vi "FRC Create Project.vi"(0 "Project folder":path, 1 "Project name":string, 2 "Team number":string, 3 "error in":errorcluster, 4 "frc project type":T1) -> (5 "proceed?":bool, 6 "error out":errorcluster)   [LabVIEW 2027]
uses:
  <resource>/plugins/NewDialogFiles/ProjectWizards/FRC/frc project type.ctl
  <vilib>/Utility/Symbolic Paths/Symbolic Path ID--enum.ctl
  <resource>/plugins/NewDialogFiles/ProjectWizards/FRC/FRC Strings.vi
  <vilib>/regexp/Match Regular Expression.xnode
  <vilib>/Utility/Symbolic Paths/NI_SymbolicPaths.lvlib
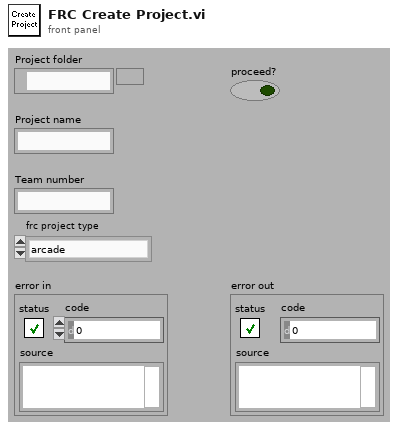
[diagram p1: front panel]
types:
  T1 = typedef "frc project type.ctl" = enum16{"arcade", "command control", "maze", "ball shooter", "dashboard", "dashboard simple", "dashboard maze", "dashboard shooter", "romi", "XRP"}
  T2 = typedef "NI_SymbolicPaths.lvlib/Symbolic Path ID--enum.ctl" = enum16{"<invalid>", "<menus>", "<vilib>", "<userlib>", "<instrlib>", "<helpdir>", "<libdir>", "<osdatadir>", "<nishared>", "<instcachedir>", "<resource>", "<extravilib>"}
  T3 = enum16{"Display", "Configure", "Hide Dialog", "Discard Ref"}
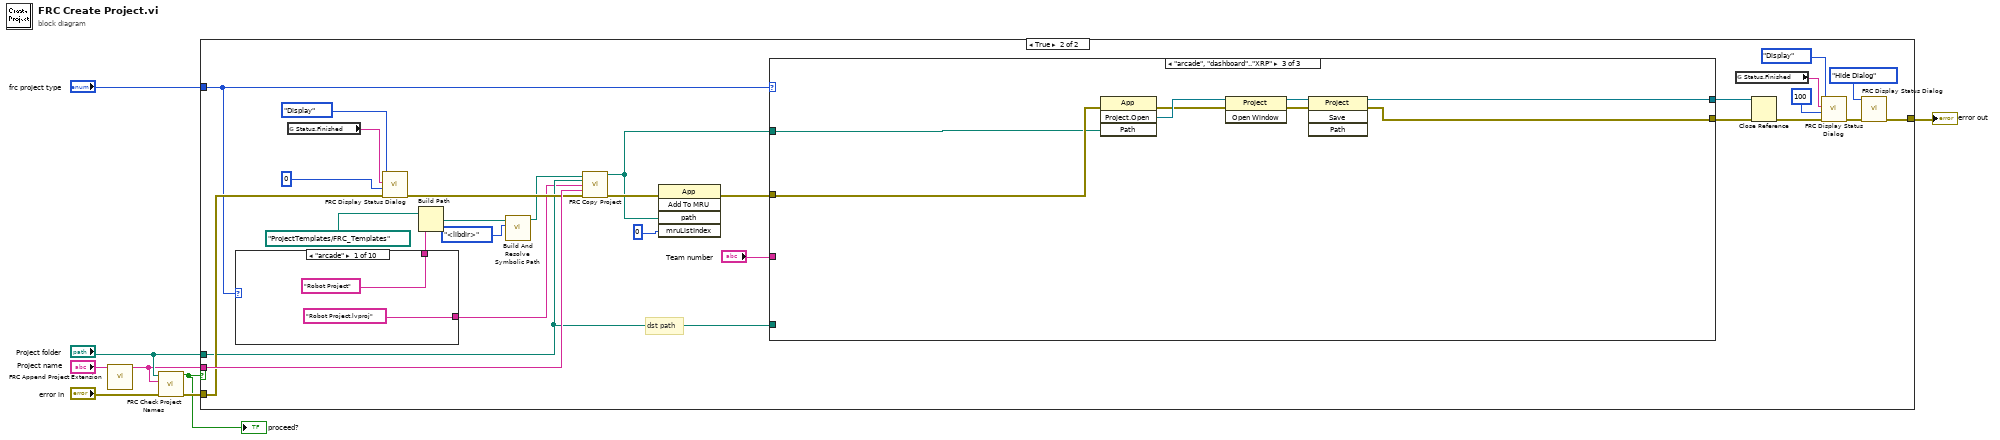
[diagram p0: block diagram]
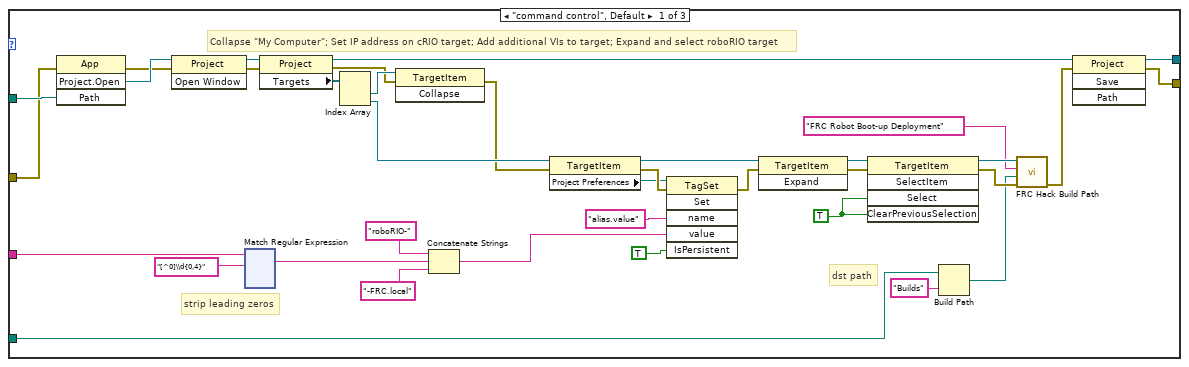
[diagram p3: hidden frame]
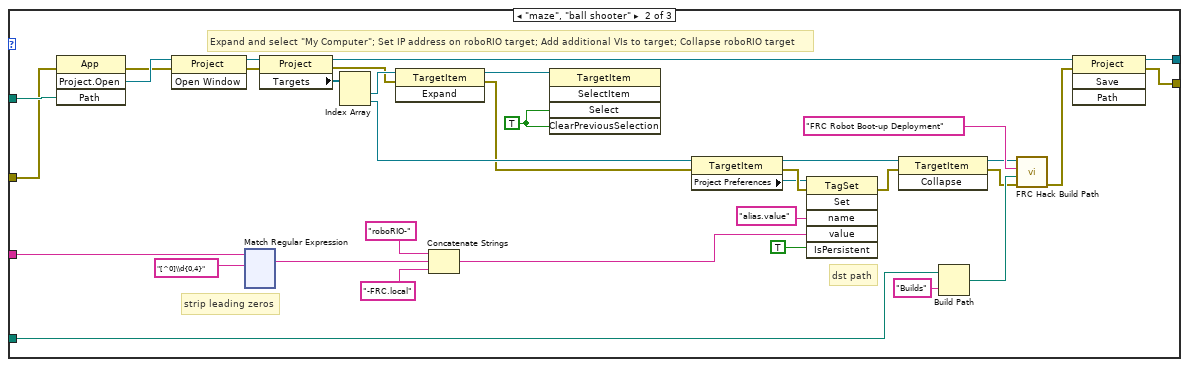
[diagram p4: hidden frame]
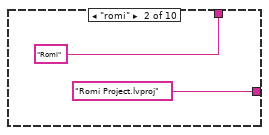
[diagram p5: hidden frame]
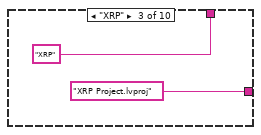
[diagram p6: hidden frame]
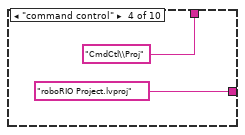
[diagram p7: hidden frame]
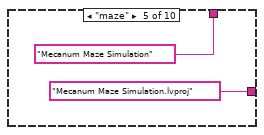
[diagram p8: hidden frame]
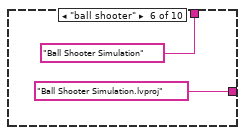
[diagram p9: hidden frame]
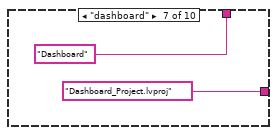
[diagram p10: hidden frame]
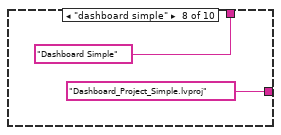
[diagram p11: hidden frame]
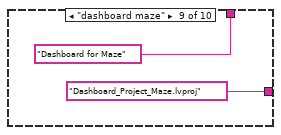
[diagram p12: hidden frame]
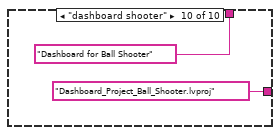
[diagram p13: hidden frame]
diagram:
  n1 = call <resource>:"FRC Append Project Extension.vi"("project name"="Project name") -> ("project name out"=w7:string)  [unwired: 1 in, 9 out]
  n2 = call <resource>:"FRC Check Project Names.vi"("error in (no error)"="error in", "project name"=w7, "project folder"="Project folder") -> ("error out"=w3:errorcluster, "proceed?"=w2:bool)  [unwired: 7 out]
  "proceed?" <- w2
  n3 = case shown="True" w2 {
    tunnel: "Project folder" -> [_ w19]
    tunnel: w7 -> [_ w37]
    tunnel: [w9 w26] -> w5
    tunnel: w3 -> [w9 w23]
    tunnel: "frc project type" -> [_ w20]
    frame False {
    }
    frame True {
      # "dst path"
      n4 = case shown="\"arcade\"" w20 {
        tunnel: ["Robot Project.lvproj" ("name or relative path") "Romi Project.lvproj" ("name or relative path") "XRP Project.lvproj" ("name or relative path") "roboRIO Project.lvproj" ("name or relative path") "Mecanum Maze Simulation.lvproj" ("name or relative path") "Ball Shooter Simulation.lvproj" ("name or relative path") "Dashboard_Project.lvproj" ("name or relative path") "Dashboard_Project_Simple.lvproj" ("name or relative path") "Dashboard_Project_Maze.lvproj" ("name or relative path") "Dashboard_Project_Ball_Shooter.lvproj" ("name or relative path")] -> w15
        tunnel: ["Robot Project" ("name or relative path") "Romi" ("name or relative path") "XRP" ("name or relative path") "CmdCtl\\Proj" ("name or relative path") "Mecanum Maze Simulation" ("name or relative path") "Ball Shooter Simulation" ("name or relative path") "Dashboard" ("name or relative path") "Dashboard Simple" ("name or relative path") "Dashboard for Maze" ("name or relative path") "Dashboard for Ball Shooter" ("name or relative path")] -> w14
        frame "arcade" {
        }
        frame "romi" {
        }
        frame "XRP" {
        }
        frame "command control" {
        }
        frame "maze" {
        }
        frame "ball shooter" {
        }
        frame "dashboard" {
        }
        frame "dashboard simple" {
        }
        frame "dashboard maze" {
        }
        frame "dashboard shooter" {
        }
      }
      n5 = global read "FRC Strings.vi" "Status.Finished"() -> (w28:string)
      n6 = call <resource>:"FRC Display Status Dialog.vi"("error in"=w23, "Numeric"=u8 0, "Text"=w28, "Mode"=T3."Display") -> ("error out"=w34:errorcluster)  [unwired: 7 out]
      n7 = Build Path(base path=path "ProjectTemplates/FRC_Templates" ("stripped path"), name or relative path=w14) -> (appended path=w11:path)
      n8 = call <vilib>:"Build And Resolve Symbolic Path.vi"("symbolic path id (<vilib>)"=Symbolic_Path_ID--enum."<libdir>" ("symbolic path id"), "relative path"=w11) -> ("resolved path"=w10:path)  [unwired: 7 in, 2 out]
      n9 = call <resource>:"FRC Copy Project.vi"("source project folder"=w10, "target path"=w19, "original project name"=w15, "new project name"=w37, "error in"=w34) -> ("new project path"=w17:path, "error out"=w36:errorcluster)  [unwired: 9 in]
      n10 = invoke class="App" method="Add To MRU"(error in=w36, "path"=w17, "mruListIndex"=0 ("Most Recently Used List Index")) -> (error out=w16:errorcluster)  [unwired: 2 in, 4 out]
      n11 = case shown="\"arcade\", \"dashboard\"..\"XRP\"" w20 {
        tunnel: [w54 w208 w348] -> w22
        tunnel: [w55 w209 w347] -> w21
        tunnel: w19 -> [w51 w206 _]
        tunnel: "Team number" -> [w43 w199 _]
        tunnel: w17 -> [w46 w202 w341]
        tunnel: w16 -> [w44 w200 w343]
        frame "command control", Default {
          w70 = TRUE ("Select")
          # "strip leading zeros"
          # "dst path"
          # "Collapse \"My Computer\"; Set IP address on cRIO target; Add additional VIs to target; Expand and select roboRIO target"
          n12 = invoke class="App" method="Project.Open"("Path"=w46) -> ("Project:Open"=w45:refnum<vi>)  [unwired: 3 in, 3 out]
          n13 = invoke class="Project" method="Open Window"(reference=w45, error in=w44) -> (reference out=w59:refnum<vi>, error out=w61:errorcluster)  [unwired: 1 in, 1 out]
          n14 = xnode "Match Regular Expression"("input string"=w43, "regular expression"="[^0]\\d{0,4}") -> ("whole match"=w38:string)  [unwired: 4 in, 4 out]
          n15 = property class="Project"(reference=w59, error in=w61) -> (reference out=w56:refnum<vi>, error out=w62:errorcluster, "Targets"=w63:refnum<vi>[])
          n16 = Index Array(array=w63) -> (element #1=w72:refnum<vi>, element #2=w71:refnum<vi>)  [unwired: 2 in]
          n17 = invoke class="TargetItem" method="Collapse"(reference=w72, error in=w62) -> (error out=w60:errorcluster)  [unwired: 1 in, 2 out]
          n18 = Concatenate Strings("roboRIO-" ("string"), w38, "-FRC.local" ("string")) -> (w42:string)
          n19 = property class="TargetItem"(reference=w71, error in=w60) -> (reference out=w58:refnum<vi>, error out=w67:errorcluster, "Project Preferences"=w64:refnum<vi>)
          n20 = invoke class="TagSet" method="Set"(reference=w64, error in=w67, "name"="alias.value" ("Name"), "value"=w42, "IsPersistent"=TRUE ("Is Persistent")) -> (error out=w57:errorcluster)  [unwired: 1 in, 5 out]
          n21 = invoke class="TargetItem" method="Expand"(reference=w58, error in=w57) -> (reference out=w68:refnum<vi>, error out=w69:errorcluster)  [unwired: 1 in, 1 out]
          n22 = invoke class="TargetItem" method="SelectItem"(reference=w68, error in=w69, "Select"=w70, "ClearPreviousSelection"=w70) -> (reference out=w49:refnum<vi>, error out=w53:errorcluster)  [unwired: 1 in, 3 out]
          n23 = Build Path(base path=w51, name or relative path="Builds") -> (appended path=w48:path)
          n24 = call <resource>:"FRC Hack Build Path.vi"("error in (no error)"=w53, "new path"=w48, "build spec name"="FRC Robot Boot-up Deployment", "TargetItem Refnum"=w49) -> ("error out"=w52:errorcluster)  [unwired: 1 in, 6 out]
          n25 = invoke class="Project" method="Save"(reference=w56, error in=w52) -> (reference out=w54:refnum<vi>, error out=w55:errorcluster)  [unwired: 2 in, 2 out]
        }
        frame "maze", "ball shooter" {
          w191 = TRUE ("Select")
          # "strip leading zeros"
          # "dst path"
          # "Expand and select \"My Computer\"; Set IP address on roboRIO target; Add additional VIs to target; Collapse roboRIO target"
          n26 = invoke class="App" method="Project.Open"("Path"=w202) -> ("Project:Open"=w201:refnum<vi>)  [unwired: 3 in, 3 out]
          n27 = invoke class="Project" method="Open Window"(reference=w201, error in=w200) -> (reference out=w213:refnum<vi>, error out=w215:errorcluster)  [unwired: 1 in, 1 out]
          n28 = xnode "Match Regular Expression"("input string"=w199, "regular expression"="[^0]\\d{0,4}") -> ("whole match"=w194:string)  [unwired: 4 in, 4 out]
          n29 = property class="Project"(reference=w213, error in=w215) -> (reference out=w210:refnum<vi>, error out=w216:errorcluster, "Targets"=w217:refnum<vi>[])
          n30 = Index Array(array=w217) -> (element #1=w223:refnum<vi>, element #2=w222:refnum<vi>)  [unwired: 2 in]
          n31 = invoke class="TargetItem" method="Expand"(reference=w223, error in=w216) -> (reference out=w190:refnum<vi>, error out=w214:errorcluster)  [unwired: 1 in, 1 out]
          n32 = Concatenate Strings("roboRIO-" ("string"), w194, "-FRC.local" ("string")) -> (w198:string)
          n33 = invoke class="TargetItem" method="SelectItem"(reference=w190, "Select"=w191, "ClearPreviousSelection"=w191) -> ()  [unwired: 2 in, 5 out]
          n34 = property class="TargetItem"(reference=w222, error in=w214) -> (reference out=w212:refnum<vi>, error out=w221:errorcluster, "Project Preferences"=w218:refnum<vi>)
          n35 = invoke class="TagSet" method="Set"(reference=w218, error in=w221, "name"="alias.value" ("Name"), "value"=w198, "IsPersistent"=TRUE ("Is Persistent")) -> (error out=w211:errorcluster)  [unwired: 1 in, 5 out]
          n36 = invoke class="TargetItem" method="Collapse"(reference=w212, error in=w211) -> (reference out=w192:refnum<vi>, error out=w193:errorcluster)  [unwired: 1 in, 1 out]
          n37 = Build Path(base path=w206, name or relative path="Builds") -> (appended path=w204:path)
          n38 = call <resource>:"FRC Hack Build Path.vi"("error in (no error)"=w193, "new path"=w204, "build spec name"="FRC Robot Boot-up Deployment", "TargetItem Refnum"=w192) -> ("error out"=w207:errorcluster)  [unwired: 1 in, 6 out]
          n39 = invoke class="Project" method="Save"(reference=w210, error in=w207) -> (reference out=w208:refnum<vi>, error out=w209:errorcluster)  [unwired: 2 in, 2 out]
        }
        frame "arcade", "dashboard".."XRP" {
          n40 = invoke class="App" method="Project.Open"(error in=w343, "Path"=w341) -> (error out=w342:errorcluster, "Project:Open"=w344:refnum<vi>)  [unwired: 2 in, 2 out]
          n41 = invoke class="Project" method="Open Window"(reference=w344, error in=w342) -> (reference out=w346:refnum<vi>, error out=w345:errorcluster)  [unwired: 1 in, 1 out]
          n42 = invoke class="Project" method="Save"(reference=w346, error in=w345) -> (reference out=w348:refnum<vi>, error out=w347:errorcluster)  [unwired: 2 in, 2 out]
        }
      }
      n43 = global read "FRC Strings.vi" "Status.Finished"() -> (w33:string)
      n44 = Close Reference(reference=w22, error in (no error)=w21) -> (error out=w24:errorcluster)
      n45 = call <resource>:"FRC Display Status Dialog.vi"("error in"=w24, "Numeric"=u8 100, "Text"=w33, "Mode"=T3."Display") -> ("error out"=w35:errorcluster)  [unwired: 7 out]
      n46 = call <resource>:"FRC Display Status Dialog.vi"("error in"=w35, "Mode"=T3."Hide Dialog") -> ("error out"=w26:errorcluster)  [unwired: 2 in, 7 out]
    }
  }
  "error out" <- w5
